vi "Save LV_data.vi"() -> ()   [LabVIEW 2020]
uses:
  LabVIEW-Python TCP Lib/LabVIEW-Python TCP Lib.lvlib
panel:
  in  "array2_name 2":T1(array[cluster])=[[{"my_name"=45.6, "my_name2"=-12, "my_bool_array"=[TRUE], "Array"=[]}]]
  out "data string":string
  in  "Cluster in 2":T2={"function_name"="do_dicf", "my_name"=1.2356, "my_name2"=0, "my_bool_array"=[FALSE, TRUE], "array2_name"=[[{"my_name"=45.6, "my_name2"=-12, "my_bool_array"=[TRUE]}]], "sin(x)"=[]}
  in  "file path (use dialog)":path=path "D:/Home/eschaub/Documents/INFORMATIQUE/LabVIEW-Python TCP/My_cluster.dat"
  out "JSON string":string="{\n  \"my_cluster_name\":{\n    \"type\":\"cluster\",\n    \"fields\":{\n      \"my_name\":{\"type\":\"DBL\"},\n      \"my_name2\":{\"type\":\"I32\"},\n      \"my_bool_array\":{\n        \"type\":\"Array\",\n        \"dimensions\":1,\n        \"element\":{\"type\":\"Boolean\"}\n      },\n      \"Array of clusters\":{\n        \"type\":\"Array\",\n        \"dimensions\":2,\n        \"element\":{\n          \"my_cluster_name\":{\n            \"type\":\"cluster\",\n            \"fields\":{\n              \"my_name\":{\"type\":\"DBL\"},\n              \"my_name2\":{\"type\":\"I32\"},\n              \"my_bool_array\":{\n                \"type\":\"Array\",\n                \"dimensions\":1,\n                \"element\":{\"type\":\"Boolean\"}\n              }\n            }\n          }\n        }\n      }\n    }\n  }\n}"
  in  "Cluster_de_depart":cluster{"fonction":string}
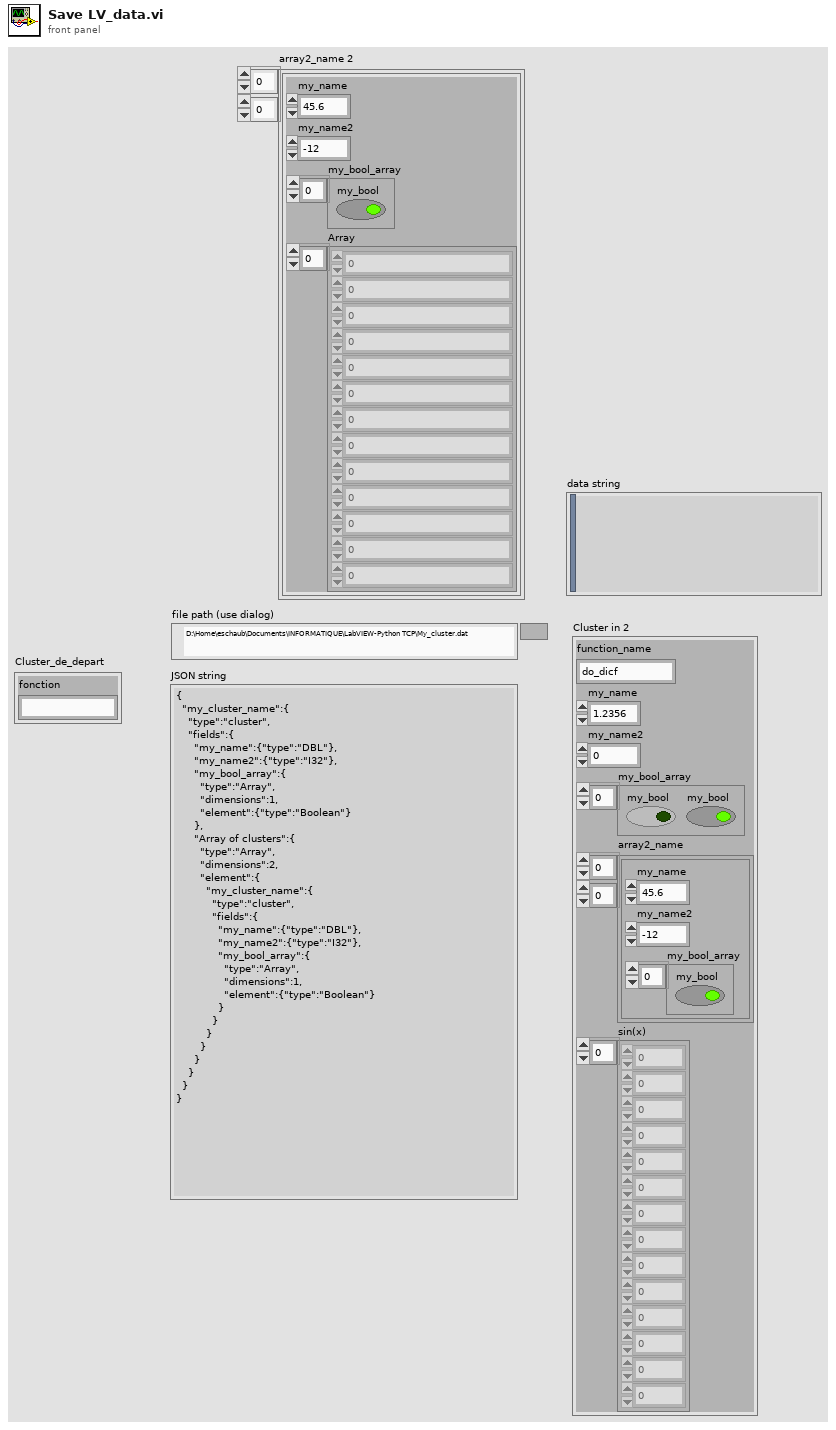
[diagram p1: front panel]
types:
  T1 = cluster{"my_name":dbl, "my_name2":i32, "my_bool_array":bool[], "Array":cdb[]}[][]
  T2 = cluster{"function_name":string, "my_name":dbl, "my_name2":i32, "my_bool_array":bool[], "array2_name":cluster{"my_name":dbl, "my_name2":i32, "my_bool_array":bool[]}[][], "sin(x)":dbl[]}
  T3 = enum16{"open", "replace", "create", "open or create", "replace or create", "replace or create with confirmation"}
  T4 = enum16{"big-endian, network order", "native, host order", "little-endian"}
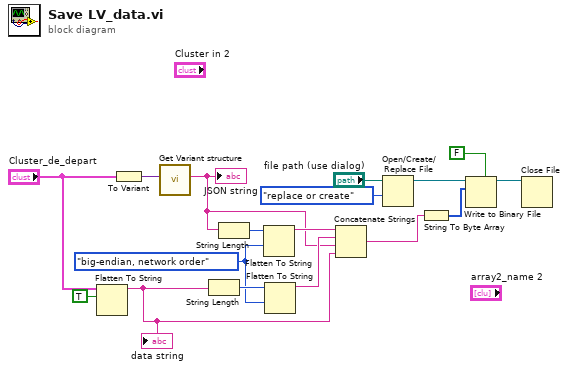
[diagram p0: block diagram]
diagram:
  w12 = T4."big-endian, network order" ("byte order (0:big-endian, network order)")
  n1 = Flatten To String(anything="Cluster_de_depart", prepend array or string size? (T)=TRUE) -> (data string=w4:string)  [unwired: 2 in, 2 out]
  "data string" <- w4
  n2 = To Variant(anything="Cluster_de_depart") -> (Variant=w1:variant)
  n3 = call "Get Variant structure.vi"("variant in"=w1) -> ("<JSON>"=w3:string)  [unwired: 10 in]
  "JSON string" <- w3
  n4 = String Length(string=w4) -> (length=w14:i32)
  n5 = String Length(string=w3) -> (length=w15:i32)
  n6 = Flatten To String(anything=w15, byte order (0:big-endian, network order)=w12) -> (data string=w16:string)  [unwired: 2 in, 2 out]
  n7 = Flatten To String(anything=w14, byte order (0:big-endian, network order)=w12) -> (data string=w13:string)  [unwired: 2 in, 2 out]
  n8 = Concatenate Strings(w16, w13, w3, w4) -> (w7:string)
  n9 = Open/Create/Replace File(file path (use dialog)="file path (use dialog)", operation (0:open)=T3."replace or create") -> (refnum out=w8:refnum<file>)  [unwired: 4 in, 2 out]
  n10 = String To Byte Array(string=w7) -> (unsigned byte array=w5:u8[])
  n11 = Write to Binary File(file (use dialog)=w8, data=w5, 5:FALSE ("prepend array or string size? (T)")) -> (refnum out=w9:refnum<file>)  [unwired: 3 in, 2 out]
  n12 = Close File(refnum=w9) -> ()  [unwired: 1 in, 2 out]
